vi "FuncVI-FileSaveSS.vi"(5 "InstanceRef":T2, 9 "arg list":T1[](array[typedef]) {"num" format="%.2f"}) -> (0 "error out":bool, 3 "result":T1 {"num" format="%.2f"})   [LabVIEW 2021]
doc: "::: CalcExpress Toolkit :::\nCopyright (c) 2000-2026 Konstantin Shifershteyn. All rights reserved."
uses:
  cetypes.llb/CalcExpress Function Argument Info.ctl
  cetypes.llb/CalcExpress Instance RefNum.ctl
panel:
  in  "max arg num":i32=6
  in  "min arg num":i32=3
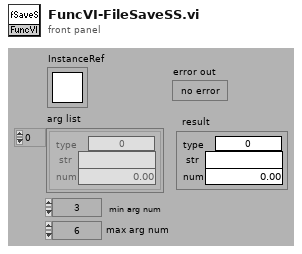
[diagram p1: front panel]
types:
  T1 = typedef "CalcExpress Function Argument Info.ctl" = cluster{"type":u32, "str":string, "num":dbl}
  T2 = typedef "CalcExpress Instance RefNum.ctl" = refnum<k1>
  T3 = enum32{"String", "DBL Number", "identifier", "1D Array of DBL", "2D Array of DBL", "CDB Number", "1D Array of CDB", "2D Array of CDB", "1D Array of String", "2D Array of String", "Unknown data type"}
  T4 = cluster{"index":i32, "data type":enum32{"String", "DBL Number", "identifier", "1D Array of DBL", "2D Array of DBL", "CDB Number", "1D Array of CDB", "2D Array of CDB", "1D Array of String", "2D Array of String", "Unknown data type"}, "default num":dbl, "default str":string}[]
  T5 = cluster{"index":i32, "any type":i32, "default num":dbl, "default str":string}
  T6 = cluster{"index":i32, "any type":u32, "default num":dbl, "default str":string}[]
  T7 = cluster{"function (open:0)":enum16{"open", "open or create", "create or replace", "create"}, "pos mode (0:2)":enum16{"start", "end", "current"}, "select mode (2)":enum32{"existing file", "new file", "new or existing file", "existing dir", "new dir", "new or existing dir", "existing file (use LLBs)", "new file (use LLBs)", "new or existing file (use LLBs)", "new or existing file or directory (use LLBs)", "existing dir (use LLBs)", "new dir (use LLBs)", "new or existing dir (use LLBs)", "existing file or dir", "new file or dir", "new or existing file or dir", "existing file or dir (use LLBs)", "new file or dir (use LLBs)"}}[]
  T8 = cluster{"function (open:0)":enum16{"open", "open or create", "create or replace", "create"}, "pos mode (0:2)":enum16{"start", "end", "current"}, "select mode (2)":enum32{"existing file", "new file", "new or existing file", "existing dir", "new dir", "new or existing dir", "existing file (use LLBs)", "new file (use LLBs)", "new or existing file (use LLBs)", "new or existing file or directory (use LLBs)", "existing dir (use LLBs)", "new dir (use LLBs)", "new or existing dir (use LLBs)", "existing file or dir", "new file or dir", "new or existing file or dir", "existing file or dir (use LLBs)", "new file or dir (use LLBs)"}}
  T9 = enum16{"open", "open or create", "create or replace", "create"}
  T10 = enum32{"existing file", "new file", "new or existing file", "existing dir", "new dir", "new or existing dir", "existing file (use LLBs)", "new file (use LLBs)", "new or existing file (use LLBs)", "new or existing file or directory (use LLBs)", "existing dir (use LLBs)", "new dir (use LLBs)", "new or existing dir (use LLBs)", "existing file or dir", "new file or dir", "new or existing file or dir", "existing file or dir (use LLBs)", "new file or dir (use LLBs)"}
  T11 = cluster{"type: use this constant to specify a predefined type code":enum32{"String", "DBL Number", "identifier", "1D Array of DBL", "2D Array of DBL", "CDB Number", "1D Array of CDB", "2D Array of CDB", "1D Array of String", "2D Array of String", "Unknown data type"}, string, "code":dbl}
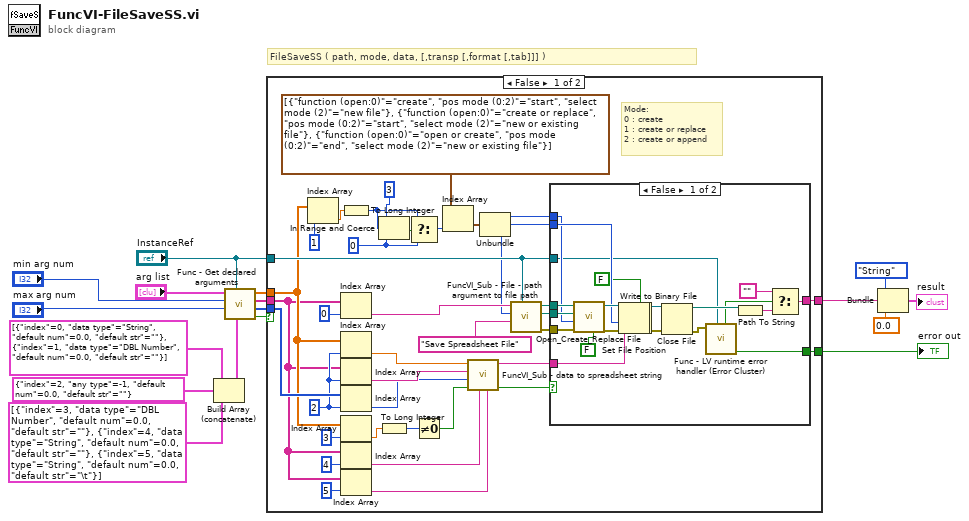
[diagram p0: block diagram]
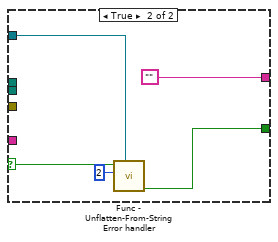
[diagram p2: hidden frame]
diagram:
  # "FileSaveSS ( path, mode, data, [,transp [,format [,tab]]] )"
  n1 = Build Array (concatenate)(T4 [{"index"=0, "data type"=enum."String", "default num"=0.0, "default str"=""}, {"index"=1, "data type"=enum."DBL Number", "default num"=0.0, "default str"=""}] ("args descriptors"), T5 {"index"=2, "any type"=-1, "default num"=0.0, "default str"=""} ("arg descriptor"), T4 [{"index"=3, "data type"=enum."DBL Number", "default num"=0.0, "default str"=""}, {"index"=4, "data type"=enum."String", "default num"=0.0, "default str"=""}, {"index"=5, "data type"=enum."String", "default num"=0.0, "default str"="\t"}] ("args descriptors")) -> (w14:T6)
  n2 = call "Func - Get declared arguments.vi"("arg descriptors"=w14, "InstanceRef"="InstanceRef", "max arg num"="max arg num", "min arg num"="min arg num", "arg list"="arg list") -> ("error out"=w11:bool, "type list"=w9:u32[], "str list"=w12:string[], "num list"=w10:dbl[])  [unwired: 3 in]
  n3 = case shown="False" w11 {
    selector: w11 -> [_ w83]
    tunnel: [w55 w83] -> w17
    tunnel: "InstanceRef" -> [w53 _]
    tunnel: w12 -> [w22 _]
    tunnel: w10 -> [w26 _]
    tunnel: w9 -> [w47 _]
    tunnel: [w18 _] -> w3
    frame False {
      w37 = 0 ("lo")
      w46 = 2
      # "Mode:\n0 : create\n1 : create or replace\n2 : create or append"
      n4 = Index Array(array=w26, index=1) -> (element=w48:dbl)
      n5 = To Long Integer(number=w48) -> (32bit integer=w35:i32)
      n6 = Index Array(array=w22, index=0) -> (element=w51:string)
      n7 = Index Array(array=w26, index=w46) -> (element=w45:dbl)
      n8 = Index Array(array=w22, index=w46) -> (element=w44:string)
      n9 = Index Array(array=w47, index=w46) -> (element=w43:u32)
      n10 = Index Array(array=w26, index=3) -> (element=w25:dbl)
      n11 = Index Array(array=w22, index=4) -> (element=w21:string)
      n12 = Index Array(array=w22, index=5) -> (element=w20:string)
      n13 = In Range and Coerce(upper limit=3 ("hi"), x=w35, lower limit=w37) -> (In Range?=w38:bool)  [unwired: 1 out]
      n14 = To Long Integer(number=w25) -> (32bit integer=w24:i32)
      n15 = Select(t=w35, s=w38, f=w37) -> (s? t:f=w34:i32)
      n16 = Not Equal To 0?(x=w24) -> (x != 0?=w23:bool)
      n17 = Index Array(array=T7 [{"function (open:0)"=enum."create", "pos mode (0:2)"=enum."start", "select mode (2)"=enum."new file"}, {"function (open:0)"=enum."create or replace", "pos mode (0:2)"=enum."start", "select mode (2)"=enum."new or existing file"}, {"function (open:0)"=enum."open or create", "pos mode (0:2)"=enum."end", "select mode (2)"=enum."new or existing file"}], index=w34) -> (element=w39:T8)
      n18 = call "FuncVI_Sub - data to spreadsheet string.vi"("delimiter (Tab)"=w20, "format string"=w21, "transpose"=w23, "data type"=w43, "flattened data"=w44, "dbl"=w45) -> ("unflatten error"=w41:bool, "spreadsheet string"=w42:string)  [unwired: 2 in]
      n19 = Unbundle(w39) -> ("function (open:0)"=w32:T9, "pos mode (0:2)"=w33:enum16{"start", "end", "current"}, "select mode (2)"=w19:T10)
      n20 = call "FuncVI_Sub - File - path argument to file path.vi"("InstanceRef"=w53, "prompt"="Save Spreadsheet File", "select mode (2)"=w19, "arg: file path"=w51) -> ("error out"=w31:errorcluster, "base path"=w50:path, "file path"=w54:path)  [unwired: 5 in]
      n21 = case shown="False" w41 {
        selector: w41 -> [_ w79]
        tunnel: [w60 w82] -> w55
        tunnel: w54 -> [w73 _]
        tunnel: w53 -> [w61 w81]
        tunnel: w50 -> [w72 _]
        tunnel: w42 -> [w70 _]
        tunnel: w33 -> [w69 _]
        tunnel: w32 -> [w68 _]
        tunnel: w31 -> [w67 _]
        tunnel: [w64 ""] -> w18
        frame False {
          n22 = call <vilib>:"Open_Create_Replace File.vi"("advisory dialog? (display:T)"=FALSE, "error in (no error)"=w67, "function (open:0)"=w68, "start path  (Not A Path)"=w72, "file path"=w73) -> ("error out"=w76:errorcluster, "refnum"=w77:refnum<file>)  [unwired: 3 in, 2 out]
          n23 = Set File Position(refnum=w77, from (0:start)=w69, error in=w76) -> (refnum out=w58:refnum<file>, error out=w57:errorcluster)  [unwired: 1 in]
          n24 = Write to Binary File(file (use dialog)=w58, data=w70, error in=w57, 5:FALSE ("prepend array or string size? (T)")) -> (refnum out=w75:refnum<file>, error out=w74:errorcluster)  [unwired: 2 in, 1 out]
          n25 = Close File(refnum=w75, error in=w74) -> (path=w66:path, error out=w62:errorcluster)
          n26 = call "Func - LV runtime error handler (Error Cluster).vi"("InstanceRef"=w61, "LabVIEW error"=w62) -> ("error out"=w60:bool, "LV error status"=w59:bool)  [unwired: 4 in, 2 out]
          n27 = Path To String(path=w66) -> (string=w65:string)
          n28 = Select(t="", s=w59, f=w65) -> (s? t:f=w64:string)
        }
        frame True {
          n29 = call "Func - Unflatten-From-String Error handler.vi"("InstanceRef"=w81, "argument number"=2, "Unflatten Error status"=w79) -> ("error out"=w82:bool)  [unwired: 6 in]
        }
      }
    }
    frame True {
    }
  }
  "error out" <- w17
  n30 = Bundle("type: use this constant to specify a predefined type code"=T3."String", w3, "code"=0.0) -> (→"result":T11)  [unwired: 1 in]
